vi "AddOrder.generated.vi"(11 "buffer.in":u64[](array[numeric])=[0, 0, 0, 0, 0, 0, 0, 0, 0]) -> (3 "OrderBook.Command":T1)   [LabVIEW 2020]
doc: "Cboe PITCH Add Order (0x21 long, 0x22 short, 0x2F expanded) -> orderbook.command: type AddOrder, orderId, side, quantity, symbol (8 chars, space padded; 6-char symbols read as 8 bytes, masked and padded so they are not byte-reversed), price (short price x100 so all prices have 4 implied decimals), nanoseconds, Add. Replaces AddOrder.vi (todo.txt items 4 and 9)."
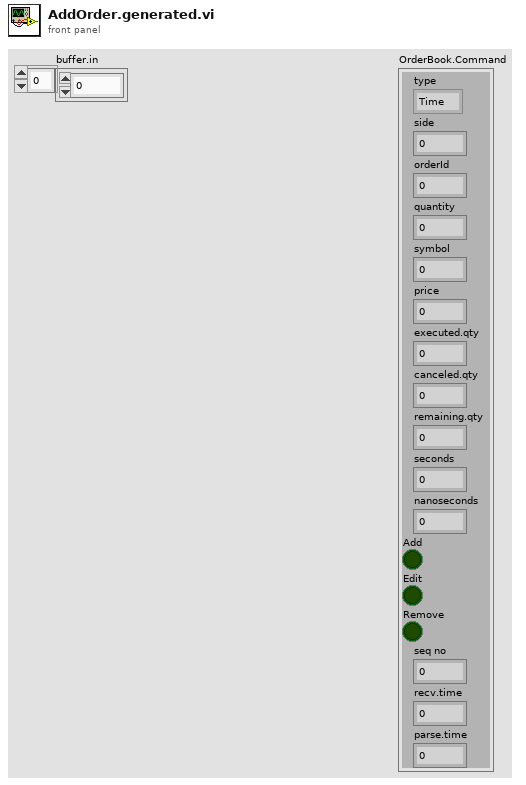
[diagram p1: front panel]
types:
  T1 = cluster{"type":enum8{"Time", "AddOrder", "OrderExecuted", "OrderExecutedAtPrice", "ReduceSize", "ModifyOrder", "DeleteOrder", "Get.Everything", "Get.All.Orders", "Get.Top", "Trade", "Unsupported"}, "side":u8, "orderId ":u64, "quantity":u32, "symbol":u64, "price":u64, "executed.qty":u32, "canceled.qty":u32, "remaining.qty":u32, "seconds":u64, "nanoseconds":u64, "Add":bool, "Edit":bool, "Remove":bool, "seq no":u32, "recv.time":u64, "parse.time":u64}
  T2 = enum8{"Time", "AddOrder", "OrderExecuted", "OrderExecutedAtPrice", "ReduceSize", "ModifyOrder", "DeleteOrder", "Get.Everything", "Get.All.Orders", "Get.Top", "Trade", "Unsupported"}
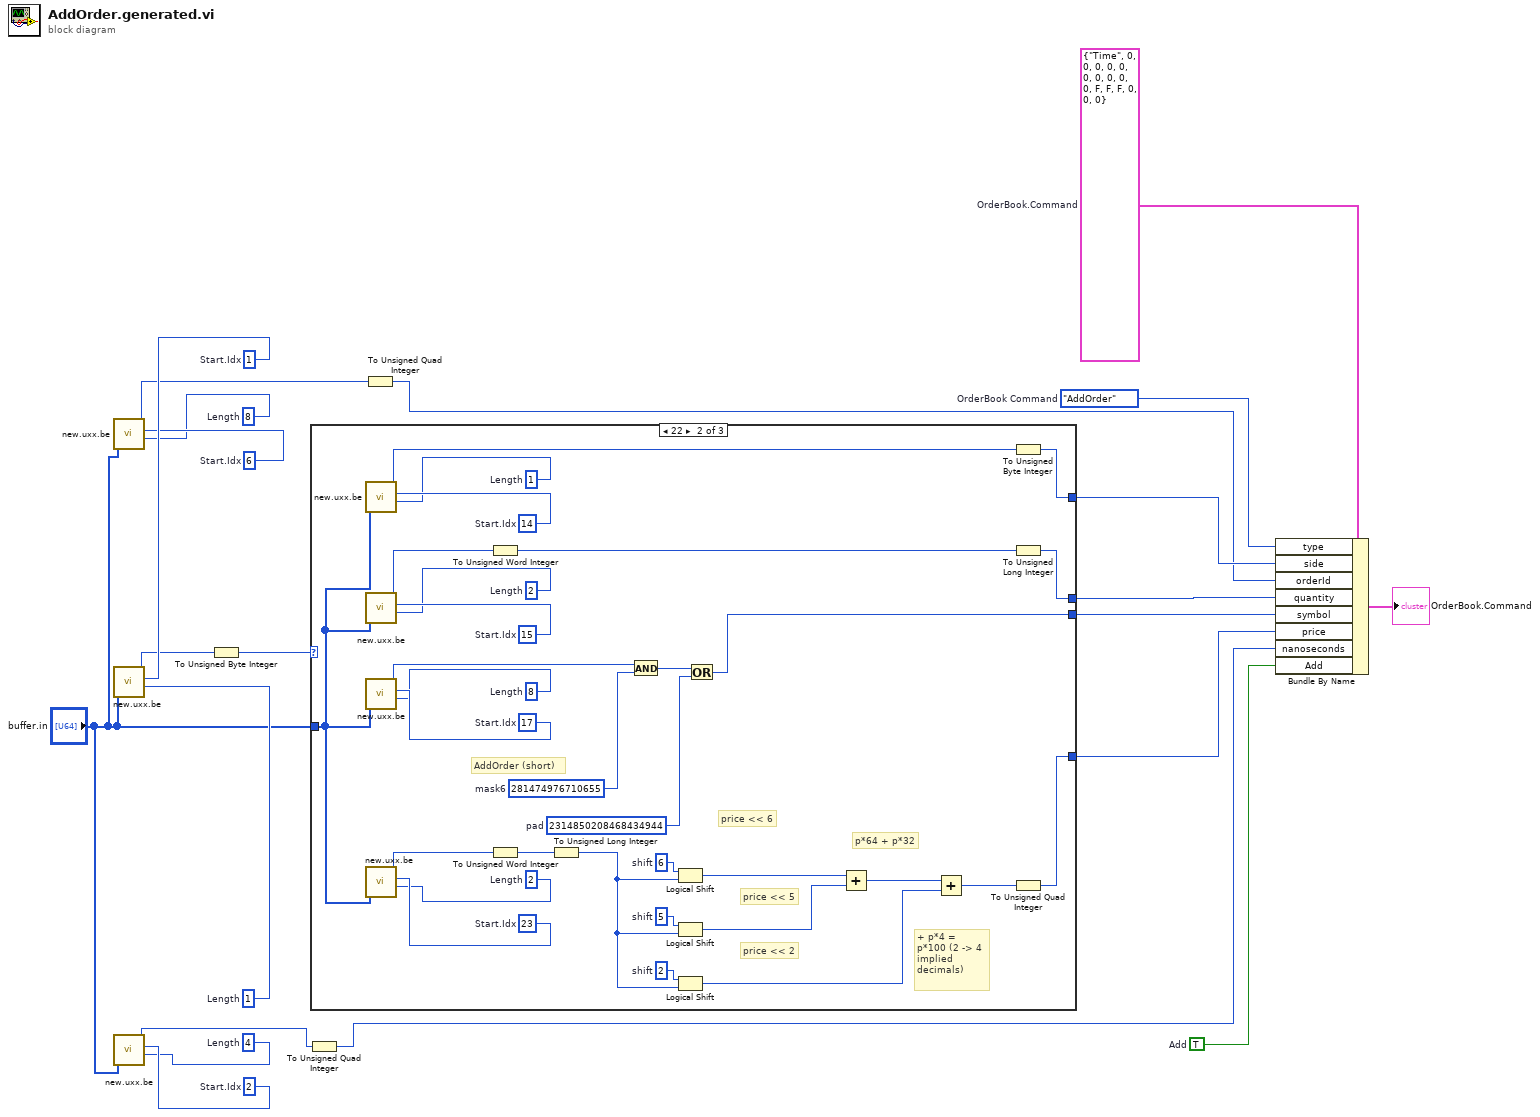
[diagram p0: block diagram]
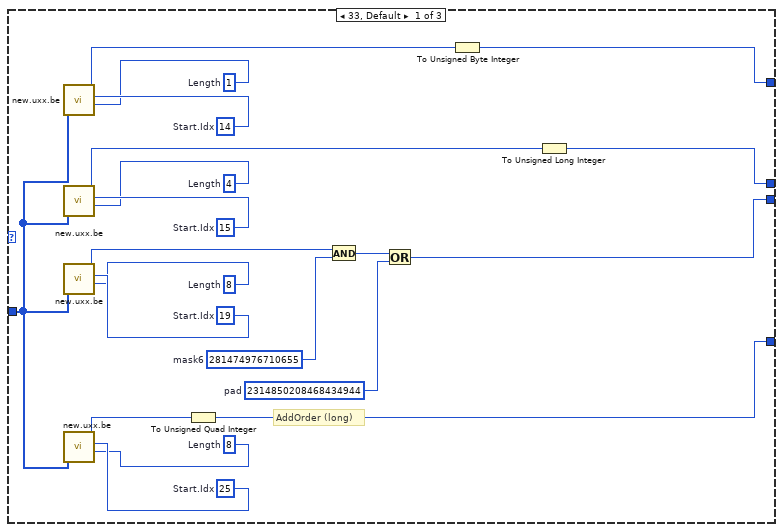
[diagram p2: hidden frame]
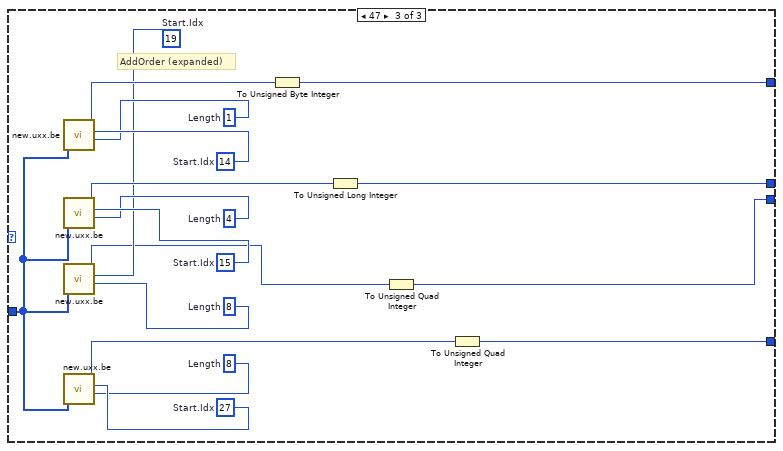
[diagram p3: hidden frame]
diagram:
  w14 = u8 8  # Length
  w15 = u8 6  # Start.Idx
  w17 = u8 4  # Length
  w18 = u8 2  # Start.Idx
  w20 = u8 1  # Length
  w21 = u8 1  # Start.Idx
  w3 = TRUE  # Add
  w10 = T2."AddOrder"  # OrderBook Command
  w2 = T1 {"type"=enum."Time", "side"=0, "orderId "=0, "quantity"=0, "symbol"=0, "price"=0, "executed.qty"=0, "canceled.qty"=0, "remaining.qty"=0, "seconds"=0, "nanoseconds"=0, "Add"=FALSE, "Edit"=FALSE, "Remove"=FALSE, "seq no"=0, "recv.time"=0, "parse.time"=0}  # OrderBook.Command
  n1 = call "new.uxx.be.vi"("buffer (U64)"="buffer.in", "Start.Idx"=w15, "Length"=w14) -> ("Out.Value U64"=w13:u64)  [unwired: 7 in]
  n2 = call "new.uxx.be.vi"("buffer (U64)"="buffer.in", "Start.Idx"=w21, "Length"=w20) -> ("Out.Value U64"=w19:u64)  [unwired: 7 in]
  n3 = call "new.uxx.be.vi"("buffer (U64)"="buffer.in", "Start.Idx"=w18, "Length"=w17) -> ("Out.Value U64"=w16:u64)  [unwired: 7 in]
  n4 = To Unsigned Byte Integer(number=w19) -> (unsigned 8bit integer=w11:u8)
  n5 = To Unsigned Quad Integer(1:w16) -> (0:w4:u64)
  n6 = case shown="22" w11 {
    tunnel: "buffer.in" -> [w29 w59 w80]
    tunnel: [w25 w45 w76] -> w9
    tunnel: [w24 w44 w75] -> w7
    tunnel: [w23 w43 w74] -> w6
    tunnel: [w22 w42 w73] -> w5
    frame 33, Default {
      w27 = u8 8  # Length
      w28 = u8 25  # Start.Idx
      w30 = u64 2314850208468434944  # pad
      w32 = u64 281474976710655  # mask6
      w34 = u8 8  # Length
      w35 = u8 19  # Start.Idx
      w37 = u8 4  # Length
      w38 = u8 15  # Start.Idx
      w40 = u8 1  # Length
      w41 = u8 14  # Start.Idx
      # "AddOrder (long)"
      n7 = call "new.uxx.be.vi"("buffer (U64)"=w29, "Start.Idx"=w41, "Length"=w40) -> ("Out.Value U64"=w39:u64)  [unwired: 7 in]
      n8 = call "new.uxx.be.vi"("buffer (U64)"=w29, "Start.Idx"=w38, "Length"=w37) -> ("Out.Value U64"=w36:u64)  [unwired: 7 in]
      n9 = call "new.uxx.be.vi"("buffer (U64)"=w29, "Start.Idx"=w35, "Length"=w34) -> ("Out.Value U64"=w33:u64)  [unwired: 7 in]
      n10 = call "new.uxx.be.vi"("buffer (U64)"=w29, "Start.Idx"=w28, "Length"=w27) -> ("Out.Value U64"=w26:u64)  [unwired: 7 in]
      n11 = To Unsigned Quad Integer(1:w26) -> (0:w22:u64)
      n12 = And(x=w33, y=w32) -> (x .and. y?=w31:u64)
      n13 = Or(x=w31, y=w30) -> (x .or. y?=w23:u64)
      n14 = To Unsigned Byte Integer(number=w39) -> (unsigned 8bit integer=w25:u8)
      n15 = To Unsigned Long Integer(number=w36) -> (unsigned 32bit integer=w24:u32)
    }
    frame 34 {
      w52 = i16 2  # shift
      w53 = i16 5  # shift
      w54 = i16 6  # shift
      w57 = u8 2  # Length
      w58 = u8 23  # Start.Idx
      w60 = u64 2314850208468434944  # pad
      w62 = u64 281474976710655  # mask6
      w64 = u8 8  # Length
      w65 = u8 17  # Start.Idx
      w68 = u8 2  # Length
      w69 = u8 15  # Start.Idx
      w71 = u8 1  # Length
      w72 = u8 14  # Start.Idx
      # "+ p*4 = p*100 (2 -> 4 implied decimals)"
      # "p*64 + p*32"
      # "price << 2"
      # "price << 5"
      # "price << 6"
      # "AddOrder (short)"
      n16 = call "new.uxx.be.vi"("buffer (U64)"=w59, "Start.Idx"=w72, "Length"=w71) -> ("Out.Value U64"=w70:u64)  [unwired: 7 in]
      n17 = call "new.uxx.be.vi"("buffer (U64)"=w59, "Start.Idx"=w69, "Length"=w68) -> ("Out.Value U64"=w67:u64)  [unwired: 7 in]
      n18 = call "new.uxx.be.vi"("buffer (U64)"=w59, "Start.Idx"=w65, "Length"=w64) -> ("Out.Value U64"=w63:u64)  [unwired: 7 in]
      n19 = call "new.uxx.be.vi"("buffer (U64)"=w59, "Start.Idx"=w58, "Length"=w57) -> ("Out.Value U64"=w56:u64)  [unwired: 7 in]
      n20 = To Unsigned Word Integer(number=w67) -> (unsigned 16bit integer=w66:u16)
      n21 = To Unsigned Word Integer(number=w56) -> (unsigned 16bit integer=w55:u16)
      n22 = To Unsigned Long Integer(number=w55) -> (unsigned 32bit integer=w51:u32)
      n23 = And(x=w63, y=w62) -> (x .and. y?=w61:u64)
      n24 = Logical Shift(y=w54, x=w51) -> (x << y=w50:u32)
      n25 = Logical Shift(y=w53, x=w51) -> (x << y=w49:u32)
      n26 = Logical Shift(y=w52, x=w51) -> (x << y=w47:u32)
      n27 = Or(x=w61, y=w60) -> (x .or. y?=w43:u64)
      n28 = Add(x=w50, y=w49) -> (x+y=w48:u32)
      n29 = Add(x=w48, y=w47) -> (x+y=w46:u32)
      n30 = To Unsigned Byte Integer(number=w70) -> (unsigned 8bit integer=w45:u8)
      n31 = To Unsigned Long Integer(number=w66) -> (unsigned 32bit integer=w44:u32)
      n32 = To Unsigned Quad Integer(1:w46) -> (0:w42:u64)
    }
    frame 47 {
      w78 = u8 8  # Length
      w79 = u8 27  # Start.Idx
      w82 = u8 8  # Length
      w83 = u8 19  # Start.Idx
      w85 = u8 4  # Length
      w86 = u8 15  # Start.Idx
      w88 = u8 1  # Length
      w89 = u8 14  # Start.Idx
      # "AddOrder (expanded)"
      n33 = call "new.uxx.be.vi"("buffer (U64)"=w80, "Start.Idx"=w89, "Length"=w88) -> ("Out.Value U64"=w87:u64)  [unwired: 7 in]
      n34 = call "new.uxx.be.vi"("buffer (U64)"=w80, "Start.Idx"=w86, "Length"=w85) -> ("Out.Value U64"=w84:u64)  [unwired: 7 in]
      n35 = call "new.uxx.be.vi"("buffer (U64)"=w80, "Start.Idx"=w83, "Length"=w82) -> ("Out.Value U64"=w81:u64)  [unwired: 7 in]
      n36 = call "new.uxx.be.vi"("buffer (U64)"=w80, "Start.Idx"=w79, "Length"=w78) -> ("Out.Value U64"=w77:u64)  [unwired: 7 in]
      n37 = To Unsigned Byte Integer(number=w87) -> (unsigned 8bit integer=w76:u8)
      n38 = To Unsigned Long Integer(number=w84) -> (unsigned 32bit integer=w75:u32)
      n39 = To Unsigned Quad Integer(1:w81) -> (0:w74:u64)
      n40 = To Unsigned Quad Integer(1:w77) -> (0:w73:u64)
    }
  }
  n41 = To Unsigned Quad Integer(1:w13) -> (0:w8:u64)
  n42 = Bundle By Name(cluster=w2, "type"=w10, "side"=w9, "orderId"=w8, "quantity"=w7, "symbol"=w6, "price"=w5, "nanoseconds"=w4, "Add"=w3) -> (→"OrderBook.Command":T1)
